vi "VIH HelpGen - Build Progress Info Window - Get Output Paths.vi"() -> (0 "CHM Path":path, 1 "HTML File paths":path[](array[path]), 2 "Common path":path)   [LabVIEW 2014]
doc: "::: VI Helpeks :::\nCopyright (c) 2000-2026 Konstantin Shifershteyn. All rights reserved."
panel:
  # "VI Helpeks\nCopyright (c) 2012-2026 Konstantin Shifershteyn"
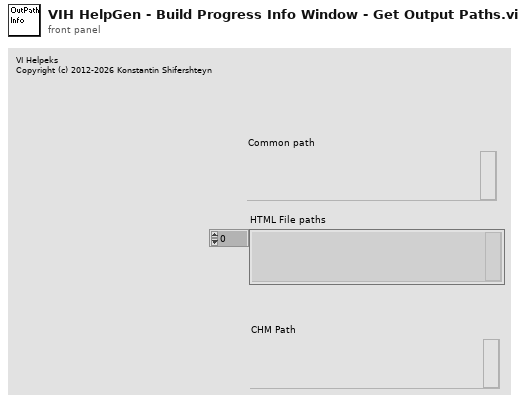
[diagram p1: front panel]
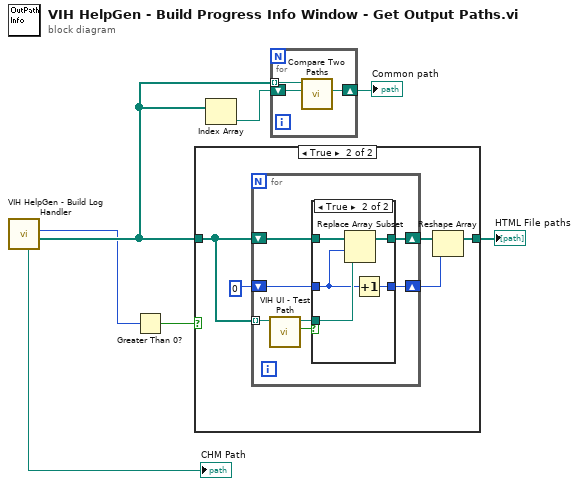
[diagram p0: block diagram]
diagram:
  n1 = call "VIH HelpGen - Build Log Handler.vi"() -> ("HTML Paths"=w4:path[], "errors"=w2:i32, "CHM Path"=→"CHM Path":path)  [unwired: 7 in, 2 out]
  n2 = Greater Than 0?(x=w2) -> (x > 0?=w3:bool)
  n3 = case shown="True" w3 {
    tunnel: w4 -> [w8 w13]
    tunnel: [w8 w9] -> w5
    frame False {
    }
    frame True {
      n4 = for {
        shift-right: [w18] -> w11
        shift-left: w13 -> [w19]
        shift-right: [w14] -> w10
        shift-left: 0 -> [w15]
        tunnel: w13 -> [w20] mode=indexing
        n5 = call "VIH UI - Test Path.vi"("Path"=w20) -> ("Good Path"=w16:bool, "dup Path"=w17:path)  [unwired: 7 in, 2 out]
        n6 = case shown="True" w16 {
          tunnel: w19 -> [w21 w27]
          tunnel: [w21 w26] -> w18
          tunnel: w17 -> [_ w25]
          tunnel: w15 -> [w22 w24]
          tunnel: [w22 w23] -> w14
          frame False {
          }
          frame True {
            n7 = Replace Array Subset(array=w27, new element=w25, index=w24) -> (w26:path[])
            n8 = Increment(x=w24) -> (x+1=w23:i32)
          }
        }
      }
      n9 = Reshape Array(w11, w10) -> (w9:path[])
    }
  }
  "HTML File paths" <- w5
  n10 = Index Array(array=w4) -> (element=w7:path)  [unwired: 1 in]
  n11 = for {
    shift-right: [w30] -> w6
    shift-left: w7 -> [w29]
    tunnel: w4 -> [w28] mode=indexing
    n12 = call <vilib>:"Compare Two Paths.vi"("Path 2"=w29, "Path 1"=w28) -> ("Common Path"=w30:path)  [unwired: 6 in, 3 out]
  }
  "Common path" <- w6
